vi "SetClientComplexityv1.vi"() -> ()   [LabVIEW 2017]
uses:
  <userlib>/_RADE/japc/classes/JSet/JSet.lvclass
panel:
  out "error out":errorcluster
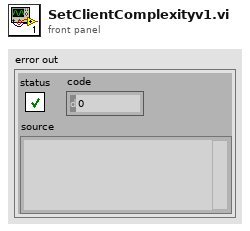
[diagram p1: front panel]
types:
  T1 = cluster{"dbl_field":dbl, "string_field":string, "long_field":i64, "int_array_field":i32[]}
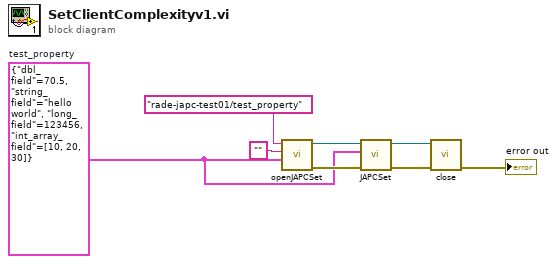
[diagram p0: block diagram]
diagram:
  w1 = T1 {"dbl_field"=70.5, "string_field"="hello world", "long_field"=123456, "int_array_field"=[10, 20, 30]}  # test_property
  n1 = call <userlib>:"openJAPCSet.vi"("Data type"=w1, "Cycle"="", "URL"="rade-japc-test01/test_property") -> ("error out"=w3:errorcluster, "Object out"=w5:refnum<class "JSet.lvclass">)  [unwired: 7 in]
  n2 = call <userlib>:"JAPCSet.vi"("error in (no error)"=w3, "Data"=w1, "Object in"=w5) -> ("error out"=w2:errorcluster, "Object out"=w4:refnum<class "JSet.lvclass">)  [unwired: 7 in]
  n3 = call-dynamic "close.vi"("error in (no error)"=w2, "Object in"=w4) -> ("error out"=→"error out":errorcluster)  [unwired: 9 in]
